vi "Actor Core.vi"(8 "error in":errorcluster, 11 "State in":refnum<class "State Actor.lvclass">) -> (0 "error out":errorcluster, 3 "Actor out":refnum<class "Actor.lvclass">)   [LabVIEW 2013, in "State Actor.lvclass"]
doc: "(<B>Filename</B>: Actor Framework.lvlib:Actor.lvclass:Actor Core.vi)\n\nThis override invokes Entry.vi on the initial state, prior to calling the parent Actor Core. Adding this behavior to Actor Core (instead of an override of Pre Launch Init.vi) allows the initial state to launch a nested actor as part of its entry behavior.\n\nReceives messages to the actor, reacts to them, and initiates any error handling that may shut the actor down.\n\nDescendant classes may override this VI to append parallel tasks for the actor to complete while it handles messages. Overrides use the Call Parent Method node."
uses:
  State Actor.lvclass
  <vilib>/ActorFramework/Actor/Actor.lvclass
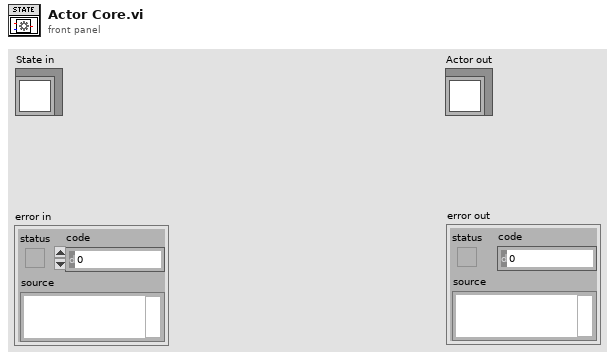
[diagram p1: front panel]
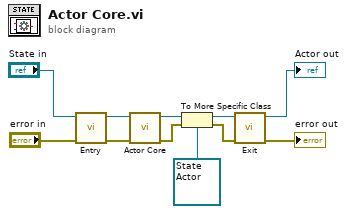
[diagram p0: block diagram]
diagram:
  n1 = call-dynamic "Entry.vi"("error in (no error)"="error in", "New State"="State in") -> ("error out"=w8:errorcluster, "State out"=w9:refnum<class "State Actor.lvclass">)  [unwired: 8 in]
  n2 = call-parent "Actor Core.vi"("error in"=w8, "Actor in"=w9) -> ("error out"=w7:errorcluster, "Actor out"=w5:refnum<class "Actor.lvclass">)  [unwired: 8 in]
  n3 = To More Specific Class(target class=refnum<class "State Actor.lvclass"> refnum ("State in"), reference=w5, error in=w7) -> (specific class reference=w4:refnum<class "State Actor.lvclass">, error out=w6:errorcluster)
  n4 = call-dynamic "Exit.vi"("error in (no error)"=w6, "Old State"=w4) -> ("error out"=→"error out":errorcluster, "New State"=→"Actor out":refnum<class "State Actor.lvclass">)  [unwired: 8 in]
